vi "UsesNi.vi"() -> (4 "bitness":string)   [LabVIEW 2026]
doc: "Test fixture: calls an NI vi.lib VI."
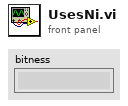
[diagram p1: front panel]
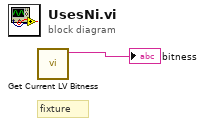
[diagram p0: block diagram]
diagram:
  # "fixture"
  n1 = call <vilib>:"Get Current LV Bitness.vi"() -> ("bitness"=→"bitness":string)  [unwired: 11 in]
